vi "Remote Exec State.vi"() -> ()   [LabVIEW 2020]
doc: "Dev helper: opens an application reference to another LabVIEW over VI Server (machine, port; e.g. LabVIEW 2020 on 3365 next to LabVIEW 2026), loads every VI listed in the items file (one path per line) there and returns per item the open error code, Execution:State as a number (0 bad = broken, 1 idle) and VI Linker Errors. Also returns that LabVIEW's version. The VIs stay in memory in that LabVIEW."
panel:
  out "error out":errorcluster
  out "linker errors":string[](array[string])
  out "states":i32[](array[numeric])
  out "codes":i32[](array[numeric])
  out "version":string
  in  "items file":path
  in  "port":u32=3365
  in  "machine":string="localhost"
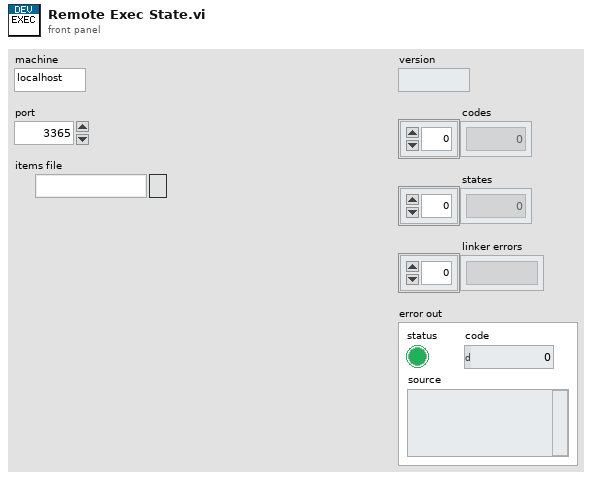
[diagram p1: front panel]
types:
  T1 = enum32{"Bad", "Idle", "Run top level", "Running"}
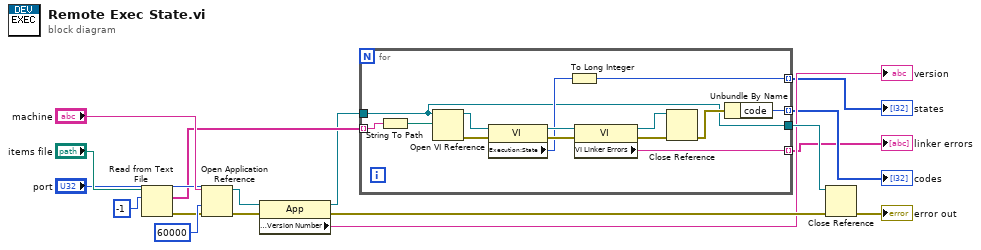
[diagram p0: block diagram]
diagram:
  n1 = Read from Text File(file (use dialog)="items file", count=-1) -> (text=w9:string[], error out=w12:errorcluster)  [unwired: 2 in, 2 out]
  n2 = Open Application Reference(8:w12, 9:60000, 10:"port", 11:"machine") -> (0:w10:errorcluster, 3:w11:refnum<vi>)
  n3 = property class="App"(reference=w11, error in=w10) -> (reference out=w8:refnum<vi>, error out=w6:errorcluster, "Application:Version Number"=→"version":string)
  n4 = for {
    tunnel: w9 -> [w31] mode=indexing
    tunnel: w8 -> [w18]
    tunnel: [w23] -> w2 mode=indexing
    tunnel: [w20] -> w4 mode=indexing
    tunnel: [w19] -> w3 mode=indexing
    tunnel: [w18] -> w7
    n5 = String To Path(string=w31) -> (path=w30:path)
    n6 = Open VI Reference(application reference (local)=w18, vi path=w30) -> (vi reference=w29:refnum<vi>, error out=w28:errorcluster)  [unwired: 4 in]
    n7 = property class="VI"(reference=w29, error in=w28) -> (reference out=w27:refnum<vi>, error out=w26:errorcluster, "Execution:State"=w22:T1)
    n8 = To Long Integer(number=w22) -> (32bit integer=w19:i32)
    n9 = property class="VI"(reference=w27, error in=w26) -> (reference out=w25:refnum<vi>, error out=w24:errorcluster, "VI Linker Errors"=w23:string)
    n10 = Close Reference(reference=w25, error in (no error)=w24) -> (error out=w21:errorcluster)
    n11 = Unbundle By Name(w21) -> ("code"=w20:i32)
  }
  "codes" <- w4
  "states" <- w3
  "linker errors" <- w2
  n12 = Close Reference(reference=w7, error in (no error)=w6) -> (error out=→"error out":errorcluster)
